vi "fake prompt name clash.vi"(10 "a_b":string, 11 "a b":string) -> (3 "prompt":string)   [LabVIEW 2020, in "MCP Server tests.lvlib"]
doc: "This is a fake prompt to test the MCP server toolkit. Its two arguments are labelled a b and a_b, which both map to the MCP name a_b, so Add Prompt.vi must refuse to register it."
uses:
  MCP Server tests.lvlib
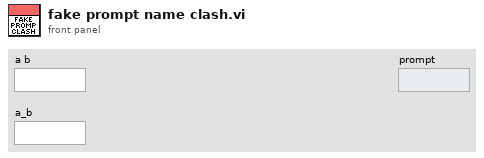
[diagram p1: front panel]
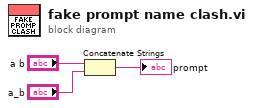
[diagram p0: block diagram]
diagram:
  n1 = Concatenate Strings("a b", "a_b") -> (→"prompt":string)
